vi "VIH Utility - FILE - Filter 1D Array of Paths.vi"(4 "Action (keep instances)":enum16{"keep instances", "remove instances"}(ring), 6 "Instances":path[](array[path]), 7 "Paths in":path[](array[path])) -> (3 "Paths out":path[](array[path]))   [LabVIEW 2014]
doc: "::: VI Helpeks :::\nCopyright (c) 2000-2026 Konstantin Shifershteyn. All rights reserved."
panel:
  # "VI Helpeks\nCopyright (c) 2012-2026 Konstantin Shifershteyn"
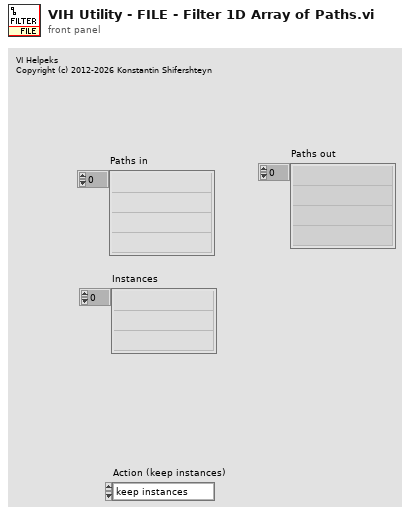
[diagram p1: front panel]
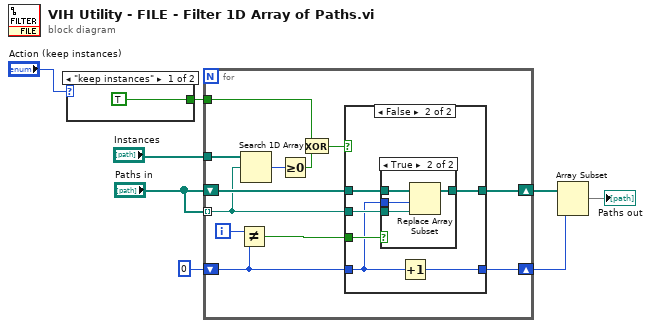
[diagram p0: block diagram]
diagram:
  n1 = case shown="\"keep instances\"" "Action (keep instances)" {
    tunnel: [TRUE _] -> w2
    frame "keep instances" {
    }
    frame "remove instances" {
    }
  }
  n2 = for {
    tunnel: "Instances" -> [w21]
    shift-right: [w17] -> w8
    shift-left: "Paths in" -> [w20]
    tunnel: "Paths in" -> [w19] mode=indexing
    shift-right: [w18] -> w1
    shift-left: 0 -> [w14]
    tunnel: w2 -> [w11]
    i -> [w15]
    n3 = Not Equal?(x=w15, y=w14) -> (x != y?=w16:bool)
    n4 = Search 1D Array(1D array=w21, element=w19) -> (index of element=w13:i32)  [unwired: 1 out]
    n5 = Greater Or Equal To 0?(x=w13) -> (x >= 0?=w12:bool)
    n6 = Exclusive Or(1:w12, 2:w11) -> (0:w10:bool)
    n7 = case shown="False" w10 {
      tunnel: w20 -> [w23 w29]
      tunnel: w19 -> [_ w28]
      tunnel: w14 -> [w22 w25]
      tunnel: [w22 w24] -> w18
      tunnel: [w23 w27] -> w17
      tunnel: w16 -> [_ w26]
      frame True {
      }
      frame False {
        n8 = case shown="True" w26 {
          tunnel: w29 -> [w30 w34]
          tunnel: w28 -> [_ w33]
          tunnel: [w30 w32] -> w27
          tunnel: w25 -> [_ w31]
          frame False {
          }
          frame True {
            n9 = Replace Array Subset(array=w34, new element=w33, index=w31) -> (w32:path[])
          }
        }
        n10 = Increment(x=w25) -> (x+1=w24:i32)
      }
    }
  }
  n11 = Array Subset(array=w8, length=w1) -> (→"Paths out":path[])  [unwired: 1 in]
